vi "upload.tdms_core.vi"(4 "Properties":map{string, string}(c390), 5 "Description":string, 7 "Name":string, 8 "error in":errorcluster, 10 "File Path":path, 11 "Nominal Client in":refnum<class "Nominal Client.lvclass">) -> (0 "error out":errorcluster, 2 "datasetRID":string, 3 "Nominal Client out":refnum<class "Nominal Client.lvclass">)   [LabVIEW 2020, in "Nominal Client.lvclass"]
doc: "Uploads a file to S3\nIngests video with common settings:\n - No TimeManifest (uses Start Timestamp and a scale factor of 1.\nNew Target: Name based on path name and timestamp"
uses:
  Nominal Client.lvclass
  datasources/dataset/dataset.lvclass
  nominal types/channelConfig/channelConfig.lvclass
  datasources/s3/s3.lvclass
  C:/code/labview-client/lv_src/datasources/source/source.lvclass
  datasources/source/create_s3.vi
  ts.epochOfTimeUnit/build.epoch.vi
  datasources/target/create_new.vi
  ingest_csv.vi
  Nominal Client.lvclass/Nominal Client.ctl
  datasources/target/target.lvclass
  datasources/source/source.lvclass
  timestampMetadata/timestampMetadata.lvclass
  ts.epochOfTimeUnit/ts.epochOfTimeUnit.lvclass
  C:/code/labview-client/lv_src/datasources/payload/payload.lvclass
  C:/code/labview-client/lv_src/datasources/s3/s3.lvclass
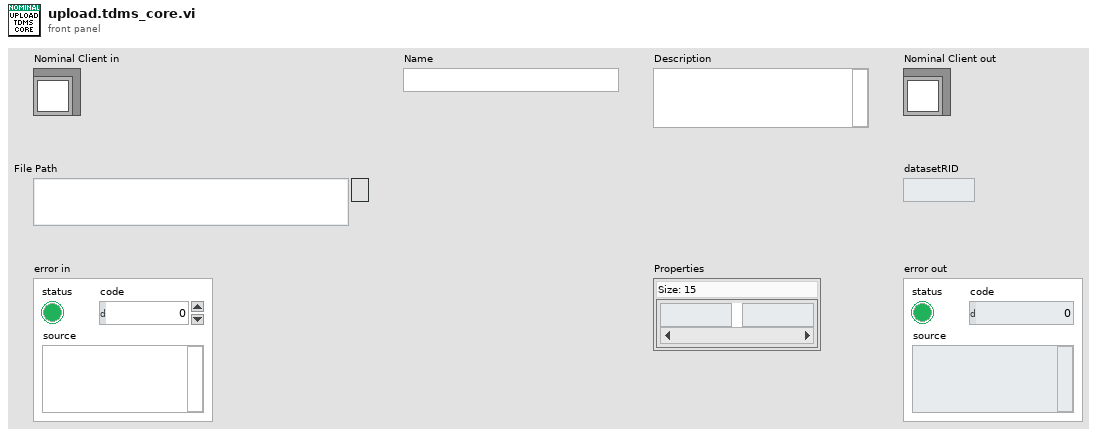
[diagram p1: front panel]
types:
  T1 = enum16{"DAYS", "HOURS", "MINUTES", "SECONDS", "MILLISECONDS", "MICROSECONDS", "NANOSECONDS", "PICOSECONDS"}
  T2 = cluster{"dataset":refnum<class "dataset.lvclass">, "channelConfig":refnum<class "channelConfig.lvclass">}
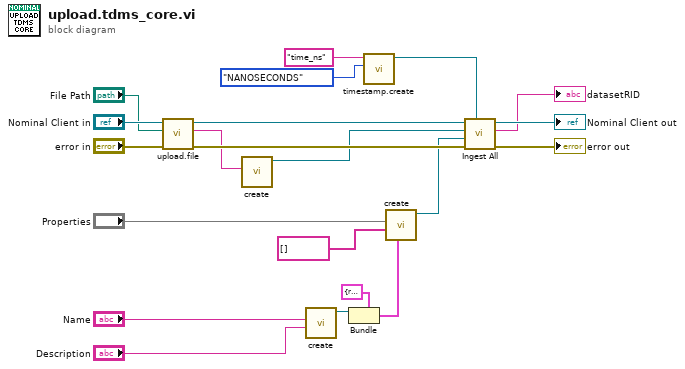
[diagram p0: block diagram]
diagram:
  n1 = call "upload.file.vi"("error in"="error in", "File"="File Path", "Nominal Client in"="Nominal Client in") -> ("error out"=w20:errorcluster, "Path to S3 File"=w18:string, "Nominal Client out"=w21:refnum<class "Nominal Client.lvclass">)  [unwired: 6 in]
  n2 = call-poly "create.vi"("Path"=w18) -> ("source"=w17:refnum<class "s3.lvclass">)  [unwired: 10 in]
  n3 = call "create.vi"("Description"="Description", "Name"="Name") -> ("dataset"=w16:refnum<class "dataset.lvclass">)  [unwired: 9 in]
  n4 = Bundle(cluster=T2 {"dataset"=refnum, "channelConfig"=refnum} ("Optional"), "dataset"=w16) -> (w15:T2)  [unwired: 1 in]
  n5 = call-poly "timestamp.create.vi"("Time Unit"=T1."NANOSECONDS", "Time Series Name"="time_ns") -> ("Timestamp Metadata"=w4:refnum<class "timestampMetadata.lvclass">)  [unwired: 9 in]
  n6 = call-poly "create.vi"("Optional"=w15, "Labels"=string[] [], "Properties"="Properties") -> ("New Target"=w19:refnum<class "target.lvclass">)  [unwired: 8 in]
  n7 = call-poly "Ingest All.vi"("timestampMetadata"=w4, "error in"=w20, "Target"=w19, "Source"=w17, "Nominal Client in"=w21) -> ("error out"=→"error out":errorcluster, "datasetRid"=→"datasetRID":string, "Nominal Client out"=→"Nominal Client out":refnum<class "Nominal Client.lvclass">)  [unwired: 3 in, 1 out]
